vi "power-spectrum-test.vi"(9 "averaging parameters":T1={"averaging mode"=enum."No averaging", "weighting mode"=enum."Exponential", "number of averages"=10, "linear mode"=enum."One shot"}, 10 "window":T2=1 items=["None"=0, "Hanning"=1, "Hamming"=2, "Blackman-Harris"=3, "Exact Blackman"=4, "Blackman"=5, "Flat Top"=6, "4 Term B-Harris "=7, "7 Term B-Harris"=8, "Low Sidelobe"=9, "Force"=64, "Exponential"=65, "Blackman Nuttall"=11, "Triangle"=30, "Bartlett-Hanning"=31, "Bohman"=32, "Parzen"=33, "Welch"=34, "Kaiser"=60, "Dolph-Chebyshev"=61, "Gaussian"=62]) -> ()   [LabVIEW 2026, in "Unit-Test.lvlib"]
uses:
  Unit-Test.lvlib
  src/Vibration-Core/Calculations.lvlib
  <vilib>/addons/_NISVFA/_Shared subVIs/Controls/svc_Window.ctl
panel:
  out "Meas array":dbl[][](array[numeric])=[[0.20093016980476444, 2.135490685983251, 0.9999894705428451, 0.46827152050181703], [0.20093016980476444, 2.135490685983251, 0.9999894705428451, 0.46827152050181703], [0.20093016980476444, 2.135490685983251, 0.9999894705428451, 0.46827152050181703]]
  out "Input Signal":waveform(dbl)[](graph)=[{"t0"=timestamp(3873836766.2642326 s since 1904-01-01), "dt"=2.0833333333333333e-05, "Y"=array[1000 elements], "attributes"=variant("Offset"=variant(dbl 0.0))}, {"t0"=timestamp(3873836766.2642326 s since 1904-01-01), "dt"=2.0833333333333333e-05, "Y"=array[1000 elements], "attributes"=variant("Offset"=variant(dbl 0.0))}, {"t0"=timestamp(3873836766.265217 s since 1904-01-01), "dt"=2.0833333333333333e-05, "Y"=array[1000 elements], "attributes"=variant("Offset"=variant(dbl 0.0))}]
  in  "frequencies [Hz] 3":dbl[](array[numeric])=[75.0, 150.0, 300.0]
  in  "frequencies [Hz] 2":dbl[](array[numeric])=[1000.0, 2000.0, 3000.0]
  in  "frequencies [Hz]":dbl[](array[numeric])=[500.0, 750.0, 900.0]
  out "Power Spectrum":cluster{"f0":dbl, "df":dbl, "magnitude":dbl[]}[](graph)=[{"f0"=0.0, "df"=48.0, "magnitude"=[2.9481009104046415e-06, 0.014300419528967604, 0.07559474229195981, 0.02629578979722698, 0.07578706649454078, 0.008067237541800113, 0.06475981822537073, 0.036306426944781735, 0.00026965844803513654, 9.588448994356172e-06, 1.181920777196556e-06, 2.517797919170074e-07, 7.401304115009457e-08, 2.6967538948334556e-08, 1.1457527341277286e-08, 5.461684479587322e-09, 2.846243632073093e-09, 1.5920809283834837e-09, 9.431616112219668e-10, 5.858208744435609e-10, 3.7857044164891074e-10, 2.5299302365968074e-10, 1.7400680226657167e-10, 1.2269884756919915e-10, 8.84221993911354e-11, 6.495287957340837e-11, 4.852993506281643e-11, 3.6813130243513523e-11, 2.8307741755703398e-11, 2.203648610451516e-11, 1.734679036776236e-11, 1.3794517681749309e-11, 1.107210765875282e-11, 8.96318238857837e-12, 7.31329161774159e-12, 6.010710368616574e-12, 4.97362063295902e-12, 4.141420632957429e-12, 3.4687472029103624e-12, 2.921309071352723e-12, 2.4729461680085237e-12, 2.1035300499800213e-12, 1.7974485643092742e-12, 1.542501039173536e-12, 1.3290850923684857e-12, 1.1495927083044292e-12, 9.9795793794723e-13, 8.693154522200678e-13, 7.597408366448391e-13, 6.660516496531224e-13, 5.856539965986838e-13, 5.164234469559252e-13, 4.566120429812303e-13, 4.047752616945356e-13, 3.597143313661655e-13, 3.2043043431220847e-13, 2.8608816316493734e-13, 2.5598622070400926e-13, 2.2953381911365247e-13, 2.0623158577289285e-13, 1.8565605014266556e-13, 1.6744698839561202e-13, 1.5129705940217048e-13, 1.3694328515684761e-13, 1.2416002228012005e-13, 1.1275314331132586e-13, 1.0255520352276914e-13, 9.342141341054894e-14, 8.522627195524183e-14, 7.786074397265265e-14, 7.122988658328509e-14, 6.525084784198192e-14, 5.985117453407456e-14, 5.496737763867403e-14, 5.0543713127493376e-14, 4.6531143231664884e-14, 4.288644929643264e-14, 3.957147243506476e-14, 3.655246199154081e-14, 3.379951543802908e-14, 3.128609567639007e-14, 2.898861433694163e-14, 2.688607125314282e-14, 2.4959741960344058e-14, 2.3192906291566396e-14, 2.1570612243602188e-14, 2.0079470148123297e-14, 1.8707472968237772e-14, 1.744383911693429e-14, 1.627887472807327e-14, 1.5203852852481075e-14, 1.4210907218228702e-14, 1.3292938759546323e-14, 1.2443533210508476e-14, 1.1656888321928004e-14, 1.0927749551130476e-14, 1.0251353093843775e-14, 9.623375390402064e-15, 9.039888294688053e-15, 8.497319237289152e-15, 7.992415745370118e-15, 7.522213833409687e-15, 7.0840098065813906e-15, 6.6753350654775025e-15, 6.293933571452531e-15, 5.937741663219777e-15, 5.604869988620709e-15, 5.29358725672908e-15, 5.002305667422973e-15, 4.729567787441881e-15, 4.474034763013985e-15, 4.234475667381716e-15, 4.009757912065376e-15, 3.798838581036252e-15, 3.6007565965737416e-15, 3.414625644952753e-15, 3.2396277499291238e-15, 3.0750074641488845e-15, 2.920066605813361e-15, 2.7741594526394112e-15, 2.6366884044149434e-15, 2.5071000231263193e-15, 2.384881433739385e-15, 2.269557038602316e-15, 2.1606855326138484e-15, 2.0578571727505473e-15, 1.9606912873844998e-15, 1.868833999259574e-15, 1.7819561434702987e-15, 1.6997513621052919e-15, 1.6219343646381624e-15, 1.5482393216850515e-15, 1.4784184057204593e-15, 1.4122404421956525e-15, 1.349489673243176e-15, 1.289964624948838e-15, 1.2334770627039056e-15, 1.179851030289499e-15, 1.128921965178565e-15, 1.080535885562662e-15, 1.034548635100281e-15, 9.90825196984303e-16, 9.492390482083393e-16, 9.096715712298262e-16, 8.72011512039273e-16, 8.361544690260343e-16, 8.020024312124952e-16, 7.694633458651161e-16, 7.38450715872026e-16, 7.088832328085578e-16, 6.806844308236143e-16, 6.537823682866688e-16, 6.281093323056013e-16, 6.036015651439138e-16, 5.80199008028674e-16, 5.578450625301763e-16, 5.364863747541538e-16, 5.160726249600124e-16, 4.965563397457609e-16, 4.778927127433205e-16, 4.600394412011095e-16, 4.42956568289673e-16, 4.2660634176197173e-16, 4.1095307920212615e-16, 3.959630416827853e-16, 3.816043168951935e-16, 3.6784671180704743e-16, 3.5466164647326867e-16, 3.4202206364240234e-16, 3.299023346691787e-16, 3.1827817899995255e-16, 3.071265840637008e-16, 2.964257338894547e-16, 2.861549388651975e-16, 2.762945709996581e-16, 2.6682600597421577e-16, 2.577315641120024e-16, 2.4899445961104993e-16, 2.405987472817177e-16, 2.32529280202499e-16, 2.2477166182209864e-16, 2.173122074165985e-16, 2.1013790368999456e-16, 2.0323637321998762e-16, 1.965958391801061e-16, 1.9020509469500735e-16, 1.8405347086303172e-16, 1.7813080771449315e-16, 1.7242743027224509e-16, 1.6693411995809897e-16, 1.61642091630513e-16, 1.56542971636642e-16, 1.5162877661155984e-16, 1.4689189151387379e-16, 1.4232505538912306e-16, 1.3792133451084492e-16, 1.3367411686655353e-16, 1.295770889544708e-16, 1.256242207427742e-16, 1.2180975346607969e-16, 1.1812818828606877e-16, 1.1457426832401536e-16, 1.111429688206616e-16, 1.0782948965725043e-16, 1.0462923801026552e-16, 1.0153782286352769e-16, 9.855104279080393e-17, 9.566487980463727e-17, 9.28754855866678e-17, 9.017917951403381e-17, 8.757243559420291e-17, 8.505187835621544e-17, 8.261427436202297e-17, 8.02565260653921e-17, 7.797566509101403e-17, 7.576884703672108e-17, 7.363334460948909e-17, 7.156654374912177e-17, 6.95659369184101e-17, 6.762911917621464e-17, 6.575378372751457e-17, 6.393771683374775e-17, 6.217879386843629e-17, 6.04749756361148e-17, 5.882430427446712e-17, 5.722490010507153e-17, 5.567495728377604e-17, 5.417274158166383e-17, 5.2716586436332663e-17, 5.130489091448463e-17, 4.993611605821982e-17, 4.860878240228332e-17, 4.732146776552913e-17, 4.6072804541519024e-17, 4.4861477343795855e-17, 4.368622107087267e-17, 4.254581837323751e-17, 4.143909801251963e-17, 4.036493263109358e-17, 3.93222373509099e-17, 3.830996750385265e-17, 3.732711729761204e-17, 3.6372718360569604e-17, 3.544583776232937e-17, 3.454557657389425e-17, 3.367106945646651e-17, 3.282148169495369e-17, 3.199600950706262e-17, 3.119387768699752e-17, 3.041433905636236e-17, 2.9656673325455977e-17, 2.8920185769135365e-17, 2.8204206290734924e-17, 2.75080888149961e-17, 2.6831209736190958e-17, 2.6172967226589026e-17, 2.55327809543711e-17, 2.4910090566936512e-17, 2.4304355088690664e-17, 2.3715052564633605e-17, 2.3141678614381398e-17, 2.258374638001511e-17, 2.2040785784658998e-17, 2.1512342536222574e-17, 2.0997977707452447e-17, 2.0497267696720144e-17, 2.000980259577119e-17, 1.9535186441446376e-17, 1.9073036637896613e-17, 1.8622983324130602e-17, 1.8184668738213362e-17, 1.7757747020096055e-17, 1.734188390835634e-17, 1.6936755805670816e-17, 1.6542049866154396e-17, 1.6157463527539152e-17, 1.5782703889162704e-17, 1.5417487659107534e-17, 1.5061540424674777e-17, 1.4714597008788783e-17, 1.4376400437052496e-17, 1.40467019226497e-17, 1.372526083896583e-17, 1.3411843790766396e-17, 1.3106225114720269e-17, 1.2808186176164316e-17, 1.2517515024709213e-17, 1.2234006538170944e-17, 1.1957461917897925e-17, 1.1687688309740823e-17, 1.1424499296693354e-17, 1.116771381370499e-17, 1.0917156433606264e-17, 1.0672657273557645e-17, 1.0434051542817464e-17, 1.02011793273438e-17, 9.973885719198173e-18, 9.752020640329622e-18, 9.535438142527699e-18, 9.323996691993488e-18, 9.117559522984796e-18, 8.915993467020937e-18, 8.719169252277975e-18, 8.526962205007336e-18, 8.339250161672844e-18, 8.155915366883097e-18, 7.976843300669445e-18, 7.801922898184997e-18, 7.631046018080921e-18, 7.464108078915534e-18, 7.301007262974614e-18, 7.141644782632589e-18, 6.985924671795004e-18, 6.833753802747959e-18, 6.6850415880528885e-18, 6.539700063362961e-18, 6.397643764110019e-18, 6.258789804756881e-18, 6.123057457843133e-18, 5.990368183359792e-18, 5.860646021553257e-18, 5.733816763572496e-18, 5.609808416132683e-18, 5.4885511602357954e-18, 5.369976736818315e-18, 5.25401919141154e-18, 5.140614114102368e-18, 5.029698916170084e-18, 4.9212128619574554e-18, 4.815096688760196e-18, 4.7112928906918616e-18, 4.609745470150709e-18, 4.51039994236476e-18, 4.413203369888186e-18, 4.318104152711841e-18, 4.225052084577644e-18, 4.1339984230891945e-18, 4.0448955500500465e-18, 3.9576972863227456e-18, 3.872358555707392e-18, 3.788835553355092e-18, 3.707085671945765e-18, 3.627067248797748e-18, 3.548739967666176e-18, 3.472064402762099e-18, 3.3970021080577935e-18, 3.323515841170766e-18, 3.2515692362557663e-18, 3.1811267731563675e-18, 3.112153972841192e-18, 3.0446172611198145e-18, 2.978483809674482e-18, 2.9137217527869904e-18, 2.8503000047446164e-18, 2.7881881918956187e-18, 2.7273568950557657e-18, 2.667777322754619e-18, 2.609421297837706e-18, 2.552261624326984e-18, 2.4962716664937744e-18, 2.4414253596860795e-18, 2.3876974686247266e-18, 2.335063276267325e-18, 2.2834986991339716e-18, 2.2329803262549555e-18, 2.183485239141548e-18, 2.134991159809394e-18, 2.0874763162917146e-18, 2.040919471667004e-18, 1.99529993196955e-18, 1.9505975786935367e-18, 1.9067926424445296e-18, 1.8638659712232276e-18, 1.821798814670225e-18, 1.7805728917580418e-18, 1.740170380263529e-18, 1.7005738714938034e-18, 1.6617664035612069e-18, 1.6237314227913867e-18, 1.5864527595635496e-18, 1.5499146120864324e-18, 1.5141016346700602e-18, 1.4789987904728993e-18, 1.4445914014105467e-18, 1.4108651509923519e-18, 1.377806120265626e-18, 1.345400675282674e-18, 1.3136354456362475e-18, 1.282497481218434e-18, 1.251974101030919e-18, 1.2220529329654586e-18, 1.192721876269423e-18, 1.1639691223508371e-18, 1.1357831354887201e-18, 1.108152758364085e-18, 1.0810668842312614e-18, 1.0545148814000575e-18, 1.0284861927629359e-18, 1.0029706431302785e-18, 9.779582668790105e-19, 9.534392659650336e-19, 9.294041292699303e-19, 9.058435790762248e-19, 8.82748500713346e-19, 8.601100304327133e-19, 8.379195217967422e-19, 8.161684493609575e-19, 7.948487102057551e-19, 7.739520769880434e-19, 7.534707195039506e-19, 7.333969144154181e-19, 7.137232002367192e-19, 6.944421812536027e-19, 6.755466973969568e-19, 6.570297734665294e-19, 6.3888452804292e-19, 6.2110430123463335e-19, 6.036825704715533e-19, 5.866129645002712e-19, 5.698892295954021e-19, 5.535053294842414e-19, 5.374553047436405e-19, 5.2173336435728625e-19, 5.063338558004697e-19, 4.91251238083874e-19, 4.764801350544924e-19, 4.620152514021108e-19, 4.478514806712225e-19, 4.339837733306776e-19, 4.2040722042323193e-19, 4.0711705894214674e-19, 3.9410860165488593e-19, 3.8137729831079684e-19, 3.6891869965043688e-19, 3.5672845563596337e-19, 3.448023445999867e-19, 3.3313621826365586e-19, 3.2172603226058883e-19, 3.105678858817687e-19, 2.996579149603599e-19, 2.889923817932296e-19, 2.7856764919498225e-19, 2.68380138055715e-19, 2.584264010137425e-19, 2.4870303523112126e-19, 2.3920676695845635e-19, 2.2993437473665893e-19, 2.2088273609921834e-19, 2.1204879977282362e-19, 2.034295983999873e-19, 1.9502224751112552e-19, 1.868239366976396e-19, 1.7883192744264577e-19, 1.710435661239293e-19, 1.6345626035464206e-19, 1.560674974860755e-19, 1.488748271837198e-19, 1.4187587173045723e-19, 1.3506833346292326e-19, 1.284499692872618e-19, 1.2201859577850823e-19, 1.15772111026563e-19, 1.0970847543371698e-19, 1.0382570427947355e-19, 9.812186317912705e-20, 9.259512287278337e-20, 8.724366016687822e-20, 8.206575742323411e-20, 7.705972485348161e-20, 7.222393092500488e-20, 6.755683632779424e-20, 6.305691628279247e-20, 5.872271998919226e-20, 5.455286766458697e-20, 5.0545999938797914e-20, 4.670084281979898e-20, 4.301614999267561e-20, 3.9490747007143314e-20, 3.6123506594806443e-20, 3.2913345249091087e-20, 2.98592480019882e-20, 2.6960226492550472e-20, 2.421536481518069e-20, 2.1623781655752896e-20, 1.9184658788697992e-20, 1.6897218061302118e-20, 1.4760724705424012e-20, 1.277450994793898e-20, 1.0937934615657853e-20, 9.250423852352622e-21, 7.711433536954939e-21, 6.32048089068055e-21, 5.077131484488192e-21, 3.980957319825034e-21, 3.0316808100537114e-21, 2.2289269697872184e-21, 1.5724782496108202e-21, 1.0621240650493377e-21, 6.977054724630234e-22, 4.790946828624295e-22]}, ...(3 in all)]
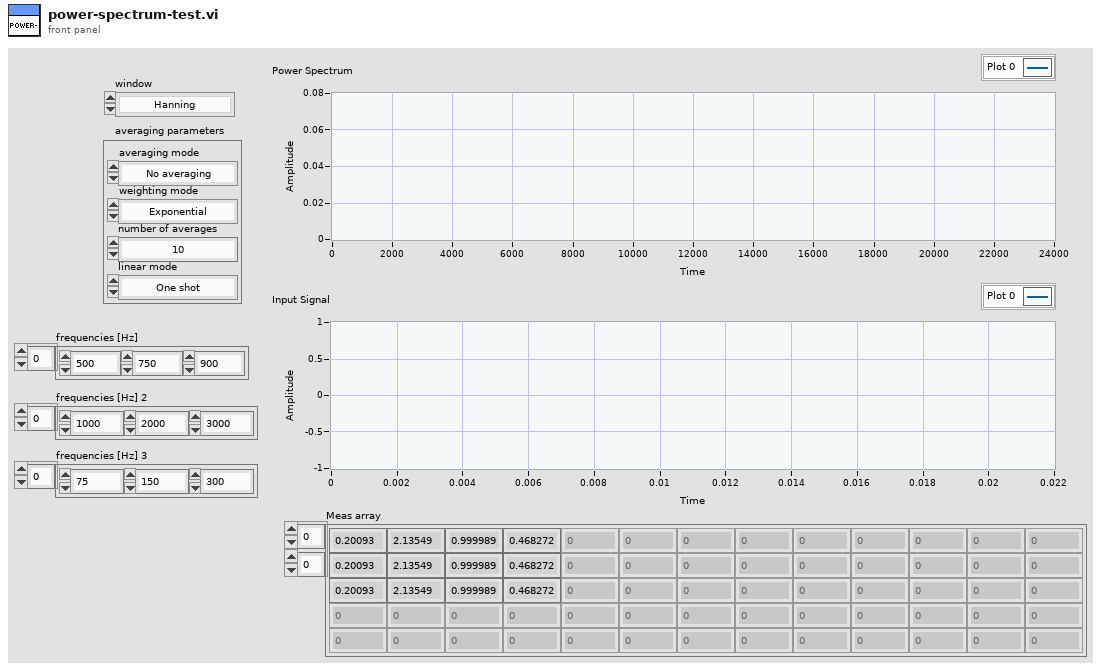
[diagram p1: front panel]
types:
  T1 = cluster{"averaging mode":enum16{"No averaging", "Vector averaging", "RMS averaging", "Peak hold"}, "weighting mode":enum16{"Linear", "Exponential"}, "number of averages":u32, "linear mode":enum16{"One shot", "Auto restart"}}
  T2 = typedef "svc_Window.ctl" = u32
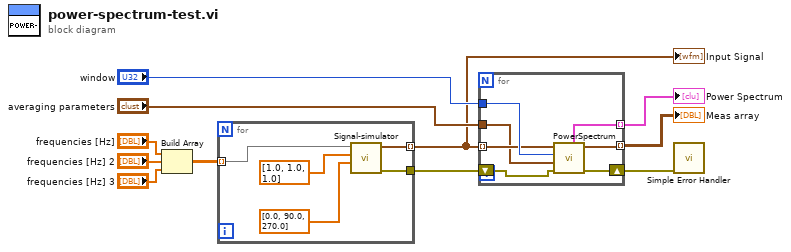
[diagram p0: block diagram]
diagram:
  n1 = Build Array("frequencies [Hz]", "frequencies [Hz] 2", "frequencies [Hz] 3") -> (w4:dbl[][])
  n2 = for {
    tunnel: [w16] -> w8
    tunnel: [w15] -> w3 mode=indexing
    tunnel: w4 -> [w14] mode=indexing
    n3 = call "Signal-simulator.vi"("phases [deg]"=dbl[] [0.0, 90.0, 270.0], "amplitudes"=dbl[] [1.0, 1.0, 1.0], "frequencies [Hz]"=w14) -> ("error out"=w16:errorcluster, "output waveform"=w15:waveform(dbl))  [unwired: 7 in]
  }
  "Input Signal" <- w3
  n4 = for {
    tunnel: [w21] -> w1 mode=indexing
    tunnel: "window" -> [w23]
    tunnel: "averaging parameters" -> [w18]
    tunnel: w3 -> [w22] mode=indexing
    shift-right: [w20] -> w9
    shift-left: w8 -> [w19]
    tunnel: [w17] -> w2 mode=indexing
    n5 = call "PowerSpectrum.vi"("error in (no error)"=w19, "averaging parameters"=w18, "Window"=w23, "Data In"=w22) -> ("error out"=w20:errorcluster, "Array of Waveforms"=w21:waveform(dbl)[], "power spectrum [dB EU]"=w17:cluster{"f0":dbl, "df":dbl, "magnitude":dbl[]})  [unwired: 5 in]
  }
  "Power Spectrum" <- w2
  "Meas array" <- w1
  n6 = call <vilib>:"Simple Error Handler.vi"("error in (no error)"=w9) -> ()  [unwired: 4 in, 5 out]
